vi "PS35_SetCalcResol.vi"(4 "error in (no error)":errorcluster, 5 "dValue":dbl=0.0001 min=0.0001 step=0.0001 format="%.5f", 6 "Axis number":i32=1 min=1 max=3, 7 "Control unit ID":i32=1 min=1 max=10) -> (0 "error out":errorcluster)   [LabVIEW 2020]
doc: "PS35_SetCalcResol.vi, created: 06.03.2009 alex; last change: 22.10.2019 alex;\n\n<B>FUNCTION:</B> \n\nSet calculated resolution for an axis.\nThe control unit uses for positioning of the axes internal values (increments).\nTo allow the positioning in other units (e.g., for the linear measuring stages - \nmm, µm, for the rotary measuring stages - degrees, mrad etc.), a calculated\nresolution per increment should be defined. Then one is able to use the \nextended functions (...Ex) with a desired unit. The specified values are \nconverted internally into increments.\nOne can use this function alternatively to the function \"PS35_SetStageAttributes\".\n----------------------------------------------------------------------------------------\n<B>INPUT:</B>\n[I32] <B>Control unit ID:</B> control unit index. (Default=1, Range=1...10) \n[I32] <B>Axis number:</B> axis number. (Default=1, Range=1...3) \n[DBL] <B>dValue:</B> resolution per increment, in desired unit. (Default=0.0001) \n[CLU] <B>error in</B>\n----------------------------------------------------------------------------------------\n<B>OUTPUT:</B>\n[CLU] <B>error out</B>\n----------------------------------------------------------------------------------------\n<B>SUB-VIs:</B>\n----------------------------------------------------------------------------------------\n<B>EXT-Calls:</B>\nps35.dll (V2.01)\n----------------------------------------------------------------------------------------"
uses:
  ps35.dll
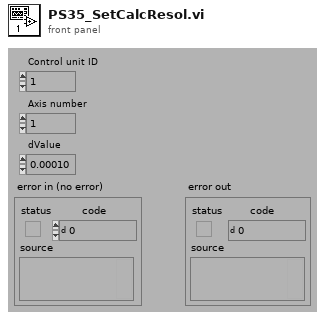
[diagram p1: front panel]
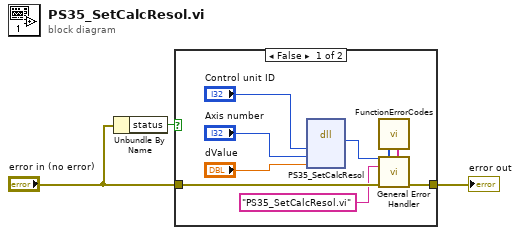
[diagram p0: block diagram]
diagram:
  n1 = Unbundle By Name("error in (no error)") -> ("status"=w1:bool)
  n2 = case shown="False" w1 {
    tunnel: "error in (no error)" -> [w11 w13]
    tunnel: [w10 w13] -> w3
    frame False {
      n3 = dll-call lib="C:/GEECS/Developers Version/source/Device Drivers/OwiSoft/OWISoftOEM/ps35/labview/lv82/ps35.dll" fn="PS35_SetCalcResol" label="PS35_Set\nCalcResol"("Index"="Control unit ID", "AxisNr"="Axis number", "dValue"="dValue") -> ("Rückgabetyp"=w9:i32)  [unwired: 6 in, 2 out]
      n4 = call "FunctionErrorCodes.vi"() -> ("[user-defined codes]"=w4:i32[], "[user-defined descriptions]"=w5:string[])  [unwired: 8 in]
      n5 = call <vilib>:"General Error Handler.vi"("[error code] (0)"=w9, "[user-defined codes]"=w4, "[user-defined descriptions]"=w5, "[error source] (\" \")"="PS35_SetCalcResol.vi" ("[error source] (\" \")"), "error in (no error)"=w11) -> ("error out"=w10:errorcluster)  [unwired: 6 in, 4 out]
    }
    frame True {
    }
  }
  "error out" <- w3
